vi "4Pi Sample Focus Control.vi"(7 "Calling VI Ref":refnum<vi>) -> ()   [LabVIEW 2021]
uses:
  4Pi Sample Focus Controls/Focus Control.ctl
  4Pi Sample Focus Controls/XY Navigation.ctl
  4Pi Sample Focus Controls/4Pi SFC - Coarse Sample Position.ctl
  <vilib>/Utility/miscctls.llb/LVPointTypeDef.ctl
  Hardware Configuration/Hardware Configuration Controls/Device Function.ctl
  Hardware Configuration/Hardware Configuration Controls/Device Type.ctl
  Device Library/Stages/Stages Controls/Stage Actions.ctl
  Device Library/Shutters/Shutter Controls/Shutter Actions.ctl
panel:
  in  "Unload Sample":bool
  in  "Coarse Sample Z Position":T1
  in  "Engage Upper Objective":bool
  in  "Toggle Shutters":bool
  in  "Lower Shutter":bool
  in  "Upper Shutter":bool
  in  "Quit":bool
  in  "Lower Objective XY":T2
  in  "Upper Objective Focus":T3 {"Step Size (µm)" format="%#_4g"}
  in  "Z Stage Focus":T3 {"Step Size (µm)" format="%#_4g"}
  # "Shutter Control"
  # "step size"
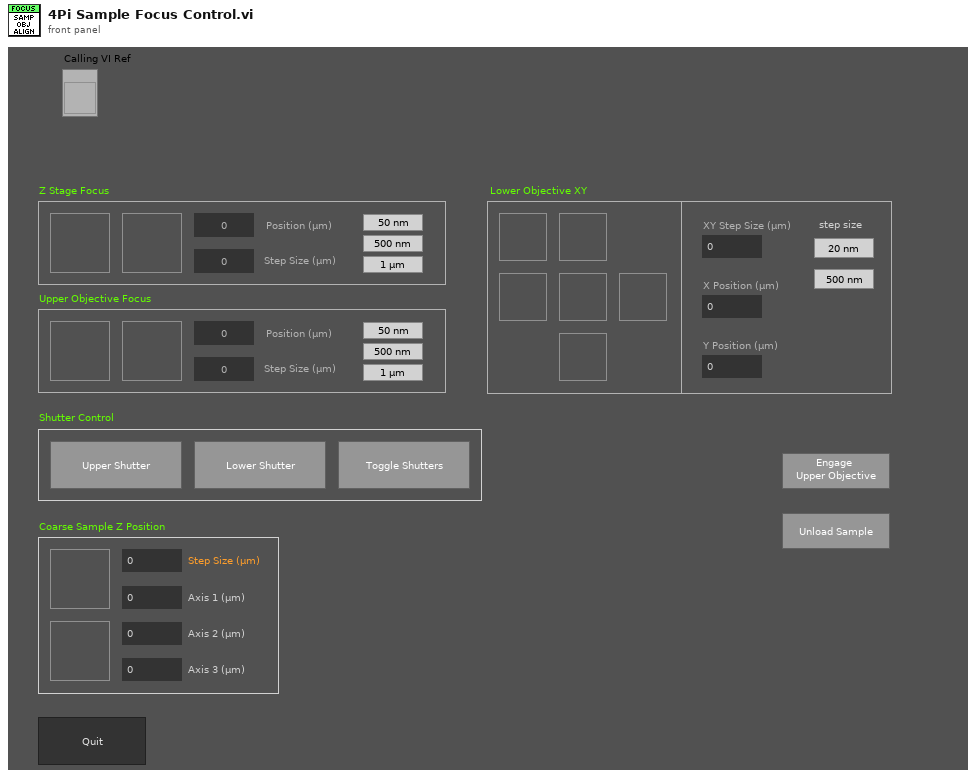
[diagram p1: front panel]
types:
  T1 = typedef "4Pi SFC - Coarse Sample Position.ctl" = cluster{"Z Up":bool, "Z Down":bool, "Step Size (µm)":dbl, "Axis 1 (µm)":dbl, "Axis 2 (µm)":dbl, "Axis 3 (µm)":dbl}
  T2 = typedef "XY Navigation.ctl" = cluster{"Up":bool, "Halt":bool, "Down":bool, "Left":bool, "Right":bool, "Home":bool, "X Position (µm)":dbl, "Y Position (µm)":dbl, "XY Step Size (µm)":dbl, "20nm step":bool, "500nm step":bool}
  T3 = typedef "Focus Control.ctl" = cluster{"Z Up":bool, "Z Down":bool, "Position (µm)":dbl, "Step Size (µm)":dbl, "50nm step":bool, "500nm step":bool, "1µm step":bool}
  T4 = enum16{"Always On", "Always Off", "Off While Running"}
  T5 = typedef "LVPointTypeDef.ctl" = cluster{"Horizontal":i16, "Vertical":i16}
  T6 = typedef "Device Function.ctl" = enum16{"Primary", "Secondary", "Overview", "Wide Field Drift Correction", "642 nm Excitation", "560 nm Excitation", "940 nm Excitation", "546 nm Excitation", "488 nm Excitation", "405 nm Excitation", "Objective Drift Correction", "4Pi Focus Lock", "4Pi Objective Lock", "Objective XY", "Objective Z", "Sample XY", "Sample Coarse Z", "Sample Z", "4Pi Lower", "4Pi Upper", "Em Small", "Em Large", "Ex Small", "Ex Large", "Mojo", "Adj Cavity", "Line Scanning", "Alert"}
  T7 = typedef "Device Type.ctl" = enum16{"AOTF", "Camera", "Deformable Mirror", "Laser", "Flip Mirror", "Shutter", "Stage", "Waveform", "FPGA", "Filter Wheel", "Email"}
  T8 = typedef "Stage Actions.ctl" = enum16{"Get Position", "SERVO OFF", "SERVO ON", "SERVO ON/OFF", "MVR", "MOVE", "HALT", "ONTARGET", "ERROR", "REFERENCE", "INIT", "VELOCITY", "STATUS", "EXIT", "HOME", "ZEROPOS", "NANOPOS", "ANALOG", "QUIT"}
  T9 = typedef "Shutter Actions.ctl" = enum16{"Open", "Close", "Toggle", "Status", "Quit"}
  T10 = cluster{"Z Up":bool, "Z Down":bool, "Position (µm)":bool, "Step Size (µm)":bool, "50nm step":bool, "500nm step":bool, "1µm step":bool}
  T11 = cluster{"Up":bool, "Halt":bool, "Down":bool, "Left":bool, "Right":bool, "Home":bool, "X Position (µm)":bool, "Y Position (µm)":bool, "XY Step Size (µm)":bool, "20nm step":bool, "500nm step":bool}
  T12 = cluster{"Z Up":bool, "Z Down":bool, "Step Size (µm)":bool, "Axis 1 (µm)":bool, "Axis 2 (µm)":bool, "Axis 3 (µm)":bool}
  T13 = typedef "LVRectTypeDef.ctl" = cluster{"Left":i16, "Top":i16, "Right":i16, "Bottom":i16}
  T14 = typedef "LVBoundsTypeDef.ctl" = cluster{"Width":u32, "Height":u32}
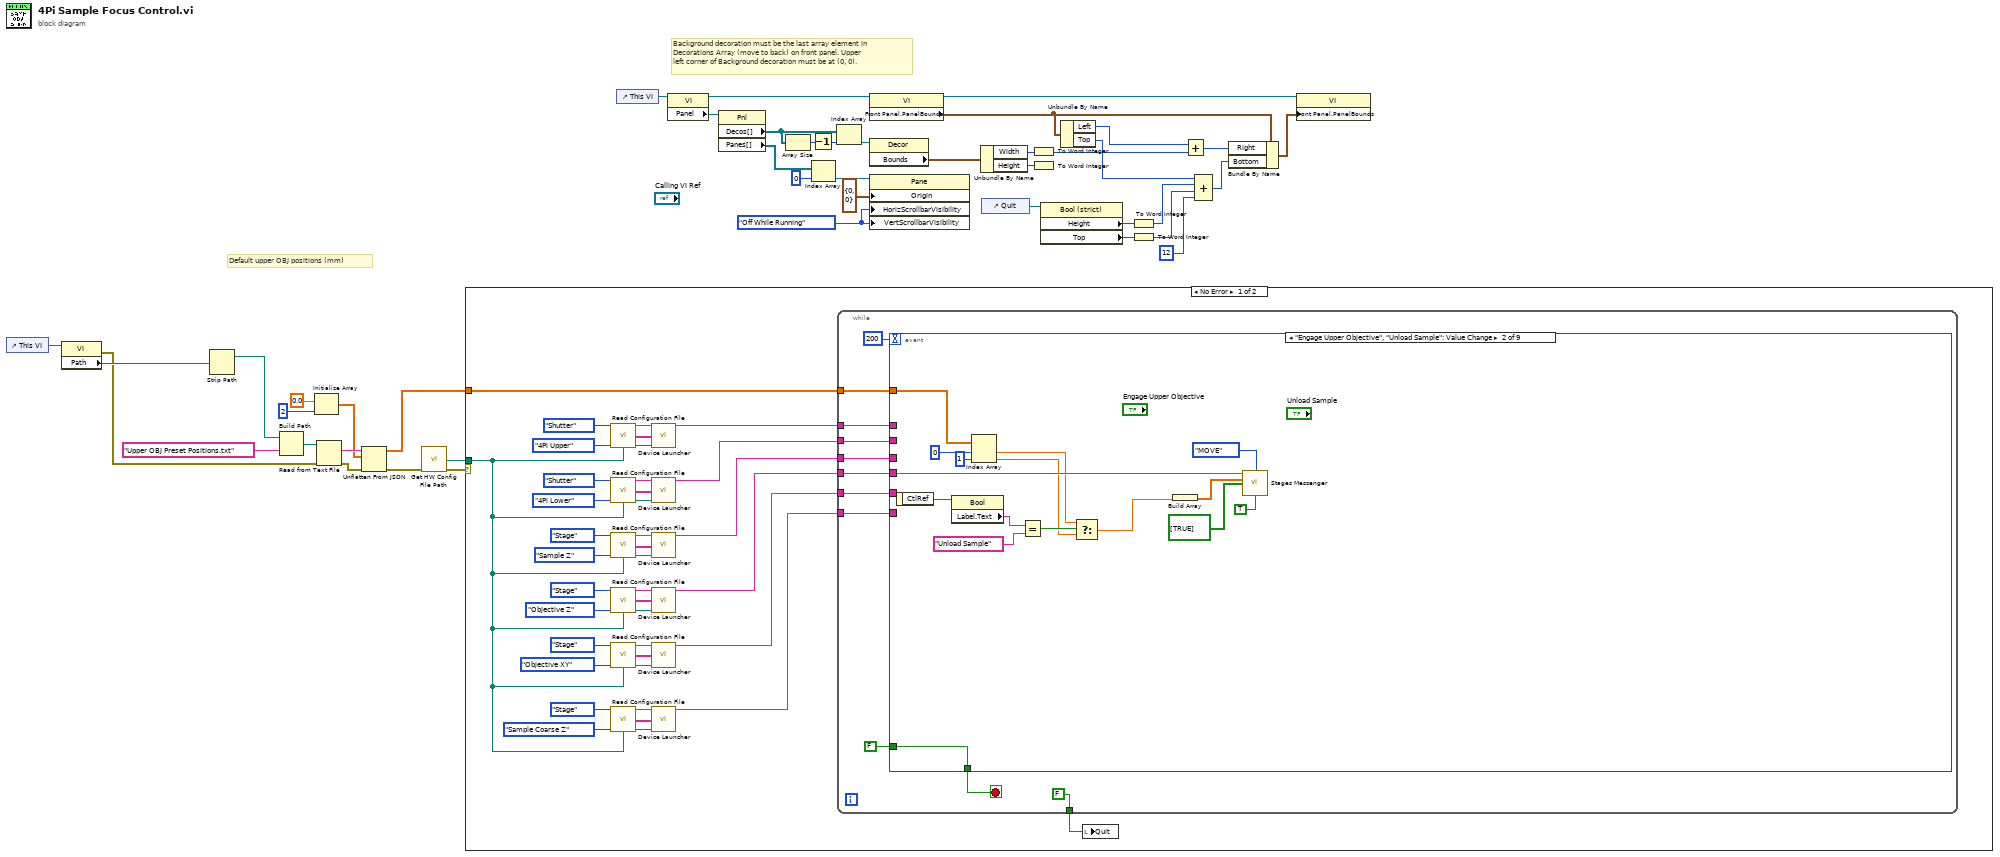
[diagram p0: block diagram]
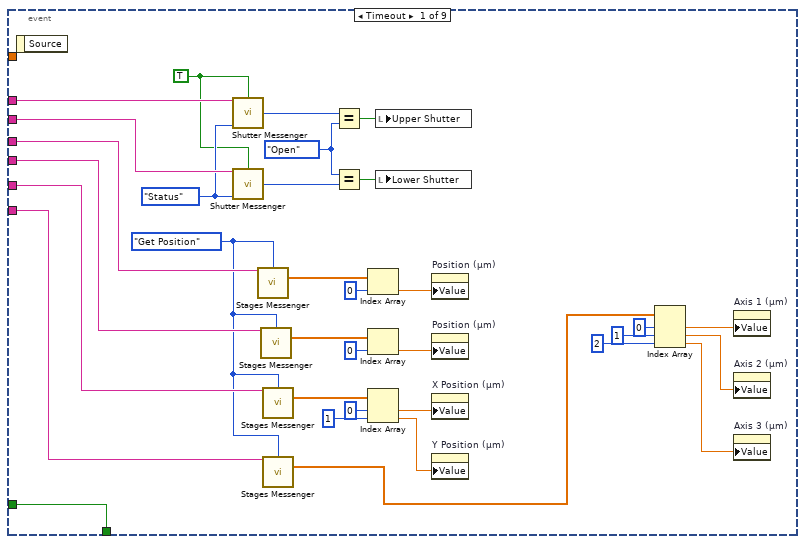
[diagram p2: hidden frame]
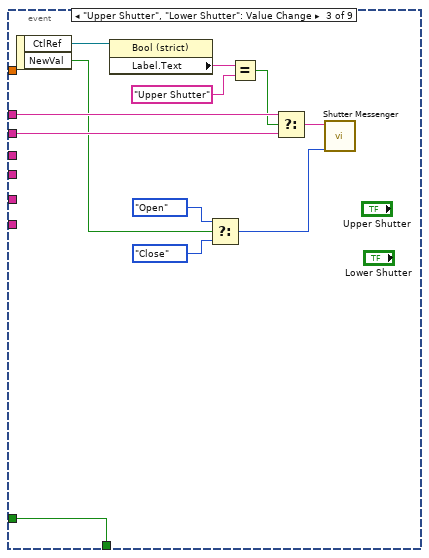
[diagram p3: hidden frame]
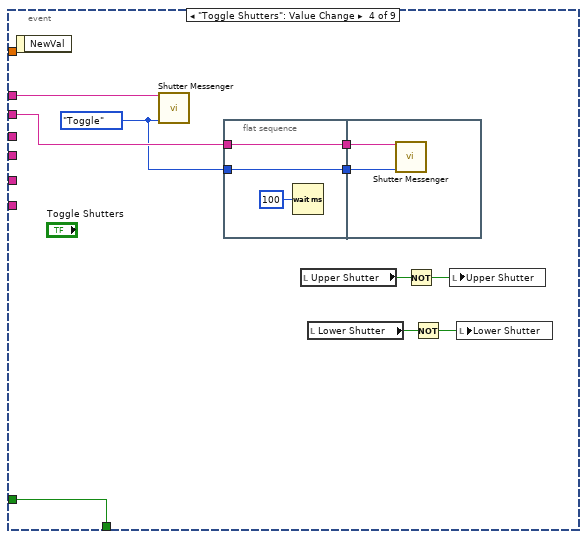
[diagram p4: hidden frame]
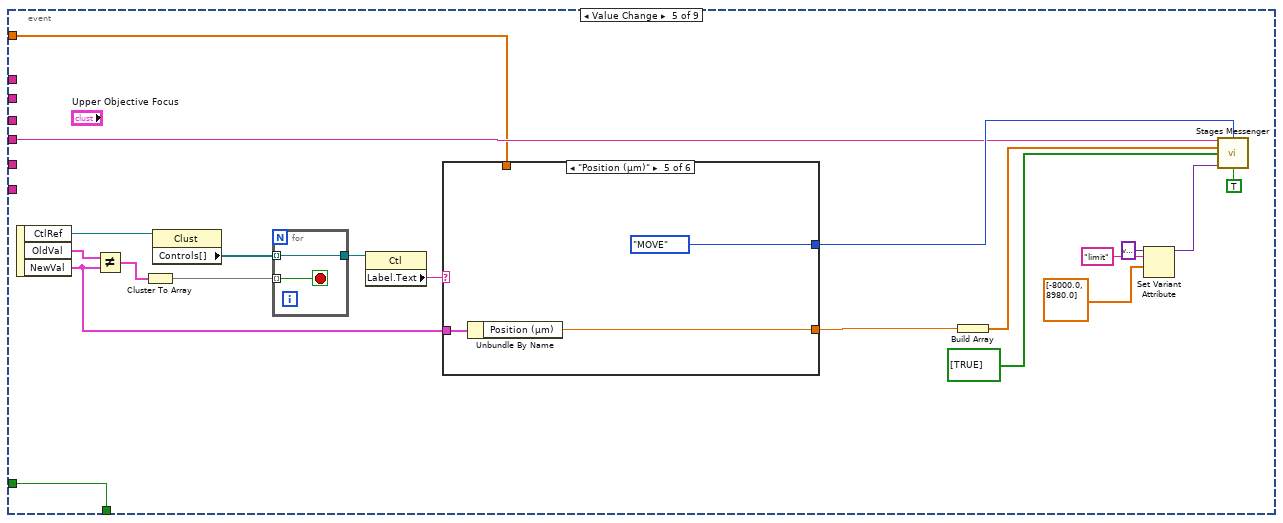
[diagram p5: hidden frame]
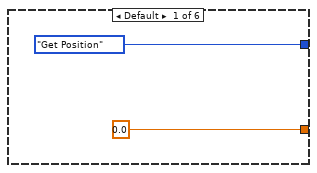
[diagram p6: hidden frame]
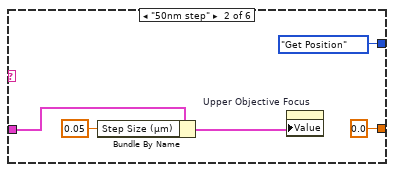
[diagram p7: hidden frame]
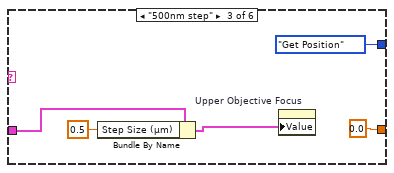
[diagram p8: hidden frame]
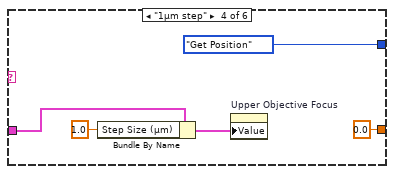
[diagram p9: hidden frame]
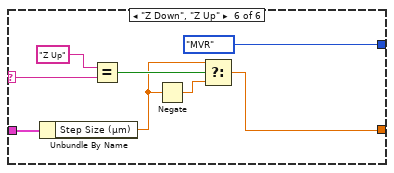
[diagram p10: hidden frame]
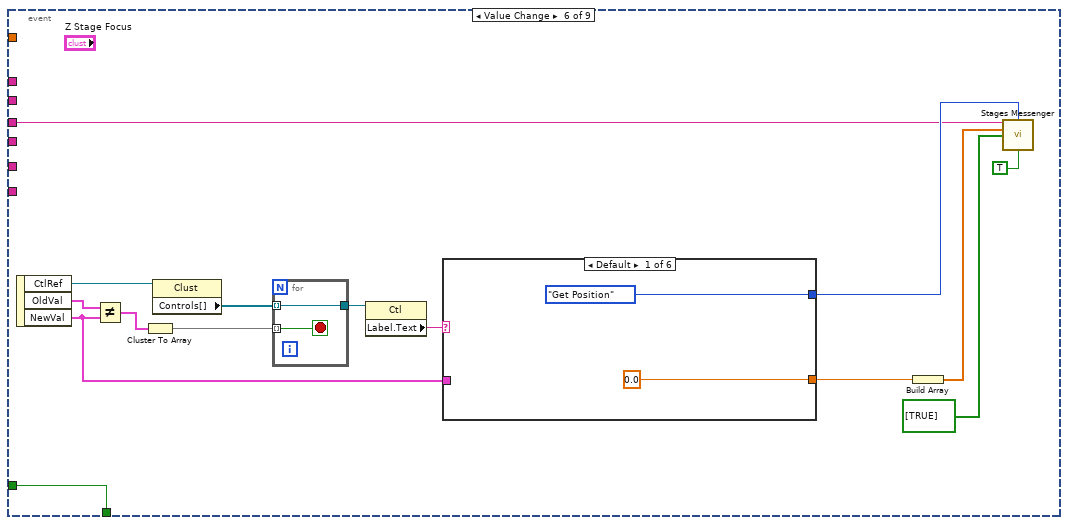
[diagram p11: hidden frame]
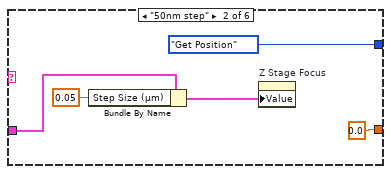
[diagram p12: hidden frame]
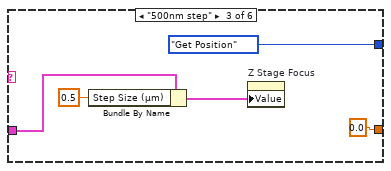
[diagram p13: hidden frame]
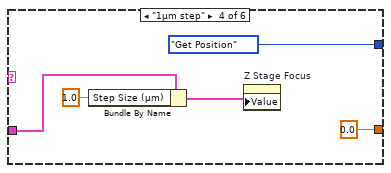
[diagram p14: hidden frame]
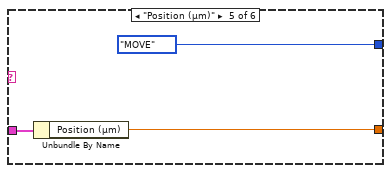
[diagram p15: hidden frame]
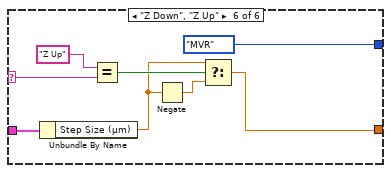
[diagram p16: hidden frame]
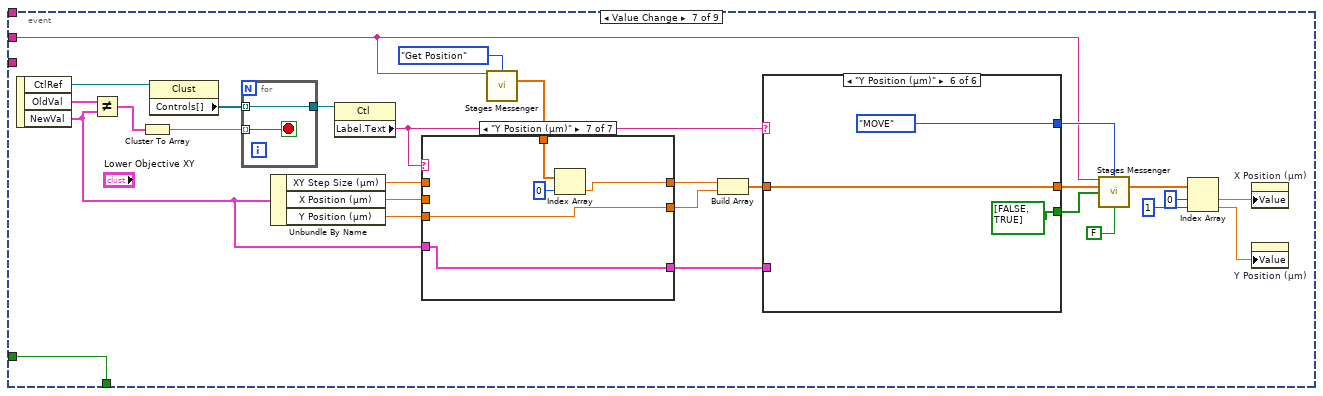
[diagram p17: hidden frame]
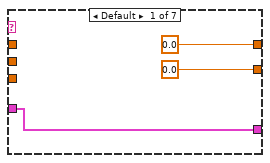
[diagram p18: hidden frame]
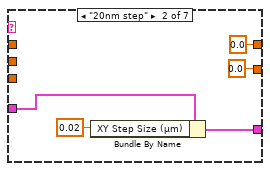
[diagram p19: hidden frame]
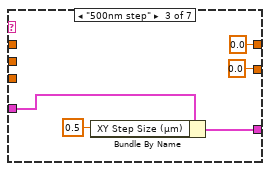
[diagram p20: hidden frame]
diagram:
  w27 = T4."Off While Running" ("Vertical Scrollbar Visibility")
  # "Default upper OBJ positions (mm)"
  # "Background decoration must be the last array element in\nDecorations Array (move to back) on front panel. Upper\nleft corner of Background decoration must be at (0, 0)."
  n1 = control-ref of="This VI"() -> (w13:refnum<vi>)
  n2 = property class="VI"(reference=w13) -> (error out=w3:errorcluster, "Path"=w12:path)  [unwired: 1 in, 1 out]
  n3 = Strip Path(path=w12) -> (stripped path=w11:path)  [unwired: 1 out]
  n4 = Build Path(base path=w11, name or relative path="Upper OBJ Preset Positions.txt") -> (appended path=w9:path)
  n5 = Initialize Array(0.0 ("element"), 2 ("dimension size")) -> (w5:dbl[])
  n6 = Read from Text File(file (use dialog)=w9, error in=w3) -> (text=w8:string, error out=w4:errorcluster)  [unwired: 2 in, 2 out]
  n7 = Unflatten From JSON(JSON string=w8, type and defaults=w5, error in (no error)=w4) -> (value=w1:dbl[], error out=w2:errorcluster)  [unwired: 4 in]
  n8 = call "Get HW Config File Path.vi"("Error"=w2) -> ("File Path"=w15:path, "Error"=w14:errorcluster)  [unwired: 13 in]
  n9 = case shown="No Error" w14 {
    tunnel: w15 -> [w47 _]
    tunnel: w1 -> [w45 _]
    frame No Error {
      n10 = call "Read Configuration File.vi"("Device Type"=Device_Type."Shutter", "Device Function"=Device_Function."4Pi Upper", "Config File Path"=w47) -> ("Unique Notifier Name"=w82:string, "Device Ports/IDs/Channels"=w81:string[], "Device Engine Path"=w80:path)  [unwired: 9 in, 1 out]
      n11 = call "Read Configuration File.vi"("Device Type"=Device_Type."Shutter", "Device Function"=Device_Function."4Pi Lower", "Config File Path"=w47) -> ("Unique Notifier Name"=w73:string, "Device Ports/IDs/Channels"=w74:string[], "Device Engine Path"=w75:path)  [unwired: 9 in, 1 out]
      n12 = call "Read Configuration File.vi"("Device Type"=Device_Type."Stage", "Device Function"=Device_Function."Sample Z", "Config File Path"=w47) -> ("Unique Notifier Name"=w61:string, "Device Ports/IDs/Channels"=w60:string[], "Device Engine Path"=w59:path)  [unwired: 9 in, 1 out]
      n13 = call "Read Configuration File.vi"("Device Type"=Device_Type."Stage", "Device Function"=Device_Function."Objective Z", "Config File Path"=w47) -> ("Unique Notifier Name"=w62:string, "Device Ports/IDs/Channels"=w63:string[], "Device Engine Path"=w64:path)  [unwired: 9 in, 1 out]
      n14 = call "Read Configuration File.vi"("Device Type"=Device_Type."Stage", "Device Function"=Device_Function."Objective XY", "Config File Path"=w47) -> ("Unique Notifier Name"=w71:string, "Device Ports/IDs/Channels"=w70:string[], "Device Engine Path"=w69:path)  [unwired: 9 in, 1 out]
      n15 = call "Read Configuration File.vi"("Device Type"=Device_Type."Stage", "Device Function"=Device_Function."Sample Coarse Z", "Config File Path"=w47) -> ("Unique Notifier Name"=w48:string, "Device Ports/IDs/Channels"=w49:string[], "Device Engine Path"=w50:path)  [unwired: 9 in, 1 out]
      n16 = call "Device Launcher.vi"("Notifier Name"=w82, "Device Ports/IDs/Channels"=w81, "Device Engine Path"=w80) -> ("Notifier Name"=w72:string)  [unwired: 11 in, 1 out]
      n17 = call "Device Launcher.vi"("Notifier Name"=w73, "Device Ports/IDs/Channels"=w74, "Device Engine Path"=w75) -> ("Notifier Name"=w83:string)  [unwired: 11 in, 1 out]
      n18 = call "Device Launcher.vi"("Notifier Name"=w61, "Device Ports/IDs/Channels"=w60, "Device Engine Path"=w59) -> ("Notifier Name"=w56:string)  [unwired: 11 in, 1 out]
      n19 = call "Device Launcher.vi"("Notifier Name"=w62, "Device Ports/IDs/Channels"=w63, "Device Engine Path"=w64) -> ("Notifier Name"=w55:string)  [unwired: 11 in, 1 out]
      n20 = call "Device Launcher.vi"("Notifier Name"=w71, "Device Ports/IDs/Channels"=w70, "Device Engine Path"=w69) -> ("Notifier Name"=w54:string)  [unwired: 11 in, 1 out]
      n21 = call "Device Launcher.vi"("Notifier Name"=w48, "Device Ports/IDs/Channels"=w49, "Device Engine Path"=w50) -> ("Notifier Name"=w46:string)  [unwired: 11 in, 1 out]
      n22 = while {
        tunnel: w72 -> [w93]
        tunnel: w83 -> [w92]
        tunnel: w56 -> [w89]
        tunnel: w55 -> [w88]
        tunnel: w54 -> [w87]
        tunnel: [FALSE] -> w53
        tunnel: w46 -> [w85]
        tunnel: w45 -> [w84]
        stop <- w90 stop-if-true
        n23 = event shown="[1] \"Engage Upper Objective\", \"Unload Sample\": Value Change" {
          selector: _ -> [_ _ _ _ _ _ _ _ _]
          dyn-events: _ -> [_ _ _ _ _ _ _ _ _]
          timeout: 200 -> [_ _ _ _ _ _ _ _ _]
          tunnel: w93 -> [w112 _ w154 w164 _ _ _ _ w410]
          tunnel: w92 -> [w111 _ w153 w163 _ _ _ _ w409]
          tunnel: FALSE -> [w127 w143 w151 w165 w190 w235 w293 w372 _]
          tunnel: [w127 w143 w151 w165 w190 w235 w293 w372 w411] -> w90
          tunnel: w89 -> [w126 _ _ _ _ w221 _ _ _]
          tunnel: w88 -> [w125 w141 _ _ w176 _ _ _ _]
          tunnel: w87 -> [w124 _ _ _ _ _ w268 _ _]
          tunnel: w85 -> [w103 _ _ _ _ _ _ w365 _]
          tunnel: w84 -> [_ w138 _ _ w175 _ _ _ _]
          event Timeout {
            w106 = Shutter_Actions."Open" ("y")
            w109 = TRUE ("Quick Status")
            w110 = Shutter_Actions."Status" ("Action")
            w102 = Stage_Actions."Get Position" ("Actions")
            n24 = event-data() -> ()  [unwired: 1 in, 1 out]
            n25 = call "Shutter Messenger.vi"("Notifier Name"=w112, "Quick Status"=w109, "Action"=w110) -> ("Shutter Status"=w108:T9)  [unwired: 11 in, 1 out]
            n26 = call "Shutter Messenger.vi"("Notifier Name"=w111, "Quick Status"=w109, "Action"=w110) -> ("Shutter Status"=w107:T9)  [unwired: 11 in, 1 out]
            n27 = call "Stages Messenger.vi"("Stage Notifier Name"=w126, "Actions"=w102) -> ("Positions"=w123:dbl[])  [unwired: 9 in, 4 out]
            n28 = call "Stages Messenger.vi"("Stage Notifier Name"=w125, "Actions"=w102) -> ("Positions"=w119:dbl[])  [unwired: 9 in, 4 out]
            n29 = call "Stages Messenger.vi"("Stage Notifier Name"=w124, "Actions"=w102) -> ("Positions"=w118:dbl[])  [unwired: 9 in, 4 out]
            n30 = call "Stages Messenger.vi"("Stage Notifier Name"=w103, "Actions"=w102) -> ("Positions"=w101:dbl[])  [unwired: 9 in, 4 out]
            n31 = Equal?(x=w108, y=w106) -> (x = y?=w105:bool)
            n32 = Equal?(x=w106, y=w107) -> (x = y?=w104:bool)
            n33 = Index Array(array=w123, index=0) -> (element=w113:dbl)
            n34 = Index Array(array=w119, index=0) -> (element=w114:dbl)
            n35 = Index Array(array=w118, index #1=0 ("index"), index #2=1 ("index")) -> (element #1=w116:dbl, element #2=w115:dbl)
            n36 = local write "Upper Shutter"(w105) -> ()
            n37 = local write "Lower Shutter"(w104) -> ()
            n38 = property on="Position (µm)" class="DigNum (strict)"("Value"=w113) -> ()  [unwired: 2 in, 2 out]
            n39 = property on="Position (µm)" class="DigNum (strict)"("Value"=w114) -> ()  [unwired: 2 in, 2 out]
            n40 = property on="X Position (µm)" class="DigNum (strict)"("Value"=w116) -> ()  [unwired: 2 in, 2 out]
            n41 = property on="Y Position (µm)" class="DigNum (strict)"("Value"=w115) -> ()  [unwired: 2 in, 2 out]
            n42 = Index Array(array=w101, index #1=0 ("index"), index #2=1 ("index"), index #3=2 ("index")) -> (element #1=w97:dbl, element #2=w96:dbl, element #3=w95:dbl)
            n43 = property on="Axis 1 (µm)" class="DigNum (strict)"("Value"=w97) -> ()  [unwired: 2 in, 2 out]
            n44 = property on="Axis 2 (µm)" class="DigNum (strict)"("Value"=w96) -> ()  [unwired: 2 in, 2 out]
            n45 = property on="Axis 3 (µm)" class="DigNum (strict)"("Value"=w95) -> ()  [unwired: 2 in, 2 out]
          }
          event "Engage Upper Objective", "Unload Sample": Value Change {
            n46 = event-data() -> ("CtlRef"=w134:refnum<vi>)  [unwired: 1 in]
            n47 = property class="Bool"(reference=w134) -> ("Label.Text"=w133:string)  [unwired: 1 in, 2 out]
            n48 = Index Array(array=w138, index #1=0 ("index"), index #2=1 ("index")) -> (element #1=w130:dbl, element #2=w128:dbl)
            n49 = Equal?(x=w133, y="Unload Sample") -> (x = y?=w131:bool)
            n50 = Select(t=w130, s=w131, f=w128) -> (s? t:f=w129:dbl)
            n51 = Build Array(w129) -> (w136:dbl[])
            n52 = call "Stages Messenger.vi"("Stage Notifier Name"=w141, "Actions"=Stage_Actions."MOVE", "Setpoint"=w136, "Axis"=bool[] [TRUE], "Exit While Busy?"=TRUE) -> ()  [unwired: 6 in, 5 out]
          }
          event "Upper Shutter", "Lower Shutter": Value Change {
            n53 = event-data() -> ("CtlRef"=w155:refnum<vi>, "NewVal"=w152:bool)  [unwired: 1 in]
            n54 = property class="Bool (strict)"(reference=w155) -> ("Label.Text"=w150:string)  [unwired: 1 in, 2 out]
            n55 = Select(t=Shutter_Actions."Open" ("Action"), s=w152, f=Shutter_Actions."Close" ("Action")) -> (s? t:f=w144:T9)
            n56 = Equal?(x=w150, y="Upper Shutter") -> (x = y?=w148:bool)
            n57 = Select(t=w154, s=w148, f=w153) -> (s? t:f=w147:string)
            n58 = call "Shutter Messenger.vi"("Notifier Name"=w147, "Action"=w144) -> ()  [unwired: 12 in, 2 out]
          }
          event "Toggle Shutters": Value Change {
            w162 = Shutter_Actions."Toggle" ("Action")
            n59 = event-data() -> ()  [unwired: 1 in, 1 out]
            n60 = call "Shutter Messenger.vi"("Notifier Name"=w164, "Action"=w162) -> ()  [unwired: 12 in, 2 out]
            n61 = flat-sequence {
              tunnel: w162 -> [w167]
              tunnel: w163 -> [w168]
              tunnel: [w168] -> w157
              tunnel: [w167] -> w156
              tunnel: w157 -> [w170]
              tunnel: w156 -> [w169]
              frame #0 {
                n62 = Wait (ms)(milliseconds to wait=u32 100) -> ()  [unwired: 1 out]
              }
              frame #1 {
                n63 = call "Shutter Messenger.vi"("Notifier Name"=w170, "Action"=w169) -> ()  [unwired: 12 in, 2 out]
              }
            }
            n64 = local read "Upper Shutter"() -> (w161:bool)
            n65 = local read "Lower Shutter"() -> (w160:bool)
            n66 = Not(x=w161) -> (.not. x?=w159:bool)
            n67 = Not(x=w160) -> (.not. x?=w158:bool)
            n68 = local write "Upper Shutter"(w159) -> ()
            n69 = local write "Lower Shutter"(w158) -> ()
          }
          event Value Change {
            n70 = event-data() -> ("CtlRef"=w189:refnum<vi>, "OldVal"=w188:T3, "NewVal"=w182:T3)  [unwired: 1 in]
            n71 = Not Equal?(x=w188, y=w182) -> (x != y?=w186:T10)
            n72 = Cluster To Array(cluster=w186) -> (array=w185:bool[])
            n73 = property class="Clust"(reference=w189) -> ("Controls[]"=w187:refnum<vi>[])  [unwired: 1 in, 2 out]
            n74 = for {
              tunnel: w187 -> [w219] mode=indexing
              tunnel: w185 -> [w220] mode=indexing
              tunnel: [w219] -> w184
              stop <- w220 stop-if-true
            }
            n75 = property class="Ctl"(reference=w184) -> ("Label.Text"=w183:string)  [unwired: 1 in, 2 out]
            n76 = case shown="\"Position (µm)\"" w183 {
              selector: w183 -> [_ _ _ _ _ w213]
              tunnel: w182 -> [_ w195 w200 w205 w209 w211]
              tunnel: [Stage_Actions."Get Position" ("Actions") Stage_Actions."Get Position" ("Actions") Stage_Actions."Get Position" ("Actions") Stage_Actions."Get Position" ("Actions") Stage_Actions."MOVE" ("Actions") Stage_Actions."MVR" ("Actions")] -> w178
              tunnel: [0.0 ("Step Size (µm)") 0.0 ("Step Size (µm)") 0.0 ("Step Size (µm)") 0.0 ("Step Size (µm)") w208 w214] -> w181
              tunnel: w175 -> [_ _ _ _ _ _]
              frame Default {
              }
              frame "50nm step" {
                n77 = Bundle By Name(cluster=w195, "Step Size (µm)"=0.05) -> (w193:T3)
                n78 = property on="Upper Objective Focus" class="Clust"("Value"=w193) -> ()  [unwired: 2 in, 2 out]
              }
              frame "500nm step" {
                n79 = Bundle By Name(cluster=w200, "Step Size (µm)"=0.5) -> (w198:T3)
                n80 = property on="Upper Objective Focus" class="Clust"("Value"=w198) -> ()  [unwired: 2 in, 2 out]
              }
              frame "1µm step" {
                n81 = Bundle By Name(cluster=w205, "Step Size (µm)"=1.0) -> (w203:T3)
                n82 = property on="Upper Objective Focus" class="Clust"("Value"=w203) -> ()  [unwired: 2 in, 2 out]
              }
              frame "Position (µm)" {
                n83 = Unbundle By Name(w209) -> ("Position (µm)"=w208:dbl)
              }
              frame "Z Down", "Z Up" {
                n84 = Unbundle By Name(w211) -> ("Step Size (µm)"=w217:dbl)
                n85 = Equal?(x="Z Up" ("t"), y=w213) -> (x = y?=w218:bool)
                n86 = Negate(x=w217) -> (-x=w216:dbl)
                n87 = Select(t=w217, s=w218, f=w216) -> (s? t:f=w214:dbl)
              }
            }
            n88 = Build Array(w181) -> (w180:dbl[])
            n89 = Set Variant Attribute(Variant=variant ("variant"), name="limit", value=dbl[] [-8000.0, 8980.0] ("Array")) -> (Variant out=w171:variant)  [unwired: 1 in, 2 out]
            n90 = call "Stages Messenger.vi"("Stage Notifier Name"=w176, "Actions"=w178, "Setpoint"=w180, "Axis"=bool[] [TRUE], "Misc"=w171, "Exit While Busy?"=TRUE) -> ()  [unwired: 5 in, 5 out]
          }
          event Value Change {
            n91 = event-data() -> ("CtlRef"=w234:refnum<vi>, "OldVal"=w233:T3, "NewVal"=w227:T3)  [unwired: 1 in]
            n92 = Not Equal?(x=w233, y=w227) -> (x != y?=w231:T10)
            n93 = Cluster To Array(cluster=w231) -> (array=w230:bool[])
            n94 = property class="Clust"(reference=w234) -> ("Controls[]"=w232:refnum<vi>[])  [unwired: 1 in, 2 out]
            n95 = for {
              tunnel: w232 -> [w264] mode=indexing
              tunnel: w230 -> [w265] mode=indexing
              tunnel: [w264] -> w229
              stop <- w265 stop-if-true
            }
            n96 = property class="Ctl"(reference=w229) -> ("Label.Text"=w228:string)  [unwired: 1 in, 2 out]
            n97 = case shown="Default" w228 {
              selector: w228 -> [_ _ _ _ _ w258]
              tunnel: w227 -> [_ w242 w247 w252 w253 w256]
              tunnel: [Stage_Actions."Get Position" ("Actions") Stage_Actions."Get Position" ("Actions") Stage_Actions."Get Position" ("Actions") Stage_Actions."Get Position" ("Actions") Stage_Actions."MOVE" ("Actions") Stage_Actions."MVR" ("Actions")] -> w223
              tunnel: [0.0 ("Step Size (µm)") 0.0 ("Step Size (µm)") 0.0 ("Step Size (µm)") 0.0 ("Step Size (µm)") w254 w259] -> w226
              frame Default {
              }
              frame "50nm step" {
                n98 = Bundle By Name(cluster=w242, "Step Size (µm)"=0.05) -> (w238:T3)
                n99 = property on="Z Stage Focus" class="Clust"("Value"=w238) -> ()  [unwired: 2 in, 2 out]
              }
              frame "500nm step" {
                n100 = Bundle By Name(cluster=w247, "Step Size (µm)"=0.5) -> (w243:T3)
                n101 = property on="Z Stage Focus" class="Clust"("Value"=w243) -> ()  [unwired: 2 in, 2 out]
              }
              frame "1µm step" {
                n102 = Bundle By Name(cluster=w252, "Step Size (µm)"=1.0) -> (w248:T3)
                n103 = property on="Z Stage Focus" class="Clust"("Value"=w248) -> ()  [unwired: 2 in, 2 out]
              }
              frame "Position (µm)" {
                n104 = Unbundle By Name(w253) -> ("Position (µm)"=w254:dbl)
              }
              frame "Z Down", "Z Up" {
                n105 = Unbundle By Name(w256) -> ("Step Size (µm)"=w262:dbl)
                n106 = Equal?(x="Z Up" ("t"), y=w258) -> (x = y?=w263:bool)
                n107 = Negate(x=w262) -> (-x=w261:dbl)
                n108 = Select(t=w262, s=w263, f=w261) -> (s? t:f=w259:dbl)
              }
            }
            n109 = Build Array(w226) -> (w225:dbl[])
            n110 = call "Stages Messenger.vi"("Stage Notifier Name"=w221, "Actions"=w223, "Setpoint"=w225, "Axis"=bool[] [TRUE], "Exit While Busy?"=TRUE) -> ()  [unwired: 6 in, 5 out]
          }
          event Value Change {
            n111 = event-data() -> ("CtlRef"=w289:refnum<vi>, "OldVal"=w288:T2, "NewVal"=w270:T2)  [unwired: 1 in]
            n112 = Not Equal?(x=w288, y=w270) -> (x != y?=w292:T11)
            n113 = Cluster To Array(cluster=w292) -> (array=w291:bool[])
            n114 = property class="Clust"(reference=w289) -> ("Controls[]"=w287:refnum<vi>[])  [unwired: 1 in, 2 out]
            n115 = for {
              tunnel: w287 -> [w357] mode=indexing
              tunnel: w291 -> [w358] mode=indexing
              tunnel: [w357] -> w290
              stop <- w358 stop-if-true
            }
            n116 = Unbundle By Name(w270) -> ("XY Step Size (µm)"=w281:dbl, "X Position (µm)"=w280:dbl, "Y Position (µm)"=w279:dbl)
            n117 = property class="Ctl"(reference=w290) -> ("Label.Text"=w282:string)  [unwired: 1 in, 2 out]
            n118 = call "Stages Messenger.vi"("Stage Notifier Name"=w268, "Actions"=Stage_Actions."Get Position") -> ("Positions"=w266:dbl[])  [unwired: 9 in, 4 out]
            n119 = case shown="\"Y Position (µm)\"" w282 {
              tunnel: w281 -> [_ _ _ w310 w315 _ _]
              tunnel: w280 -> [_ _ _ _ _ w322 _]
              tunnel: w279 -> [_ _ _ _ _ _ w327]
              tunnel: [0.0 ("Y Position (µm)") 0.0 ("X Position (µm)") 0.0 ("X Position (µm)") w309 w314 w322 w323] -> w278
              tunnel: [0.0 0.0 ("Y Position (µm)") 0.0 ("Y Position (µm)") w308 w314 w318 w327] -> w271
              tunnel: w270 -> [w294 w301 w306 w307 w313 w321 w326]
              tunnel: [w294 w297 w302 w307 w313 w321 w326] -> w269
              tunnel: w266 -> [_ _ _ _ _ w320 w325]
              frame Default {
              }
              frame "20nm step" {
                n120 = Bundle By Name(cluster=w301, "XY Step Size (µm)"=0.02) -> (w297:T2)
              }
              frame "500nm step" {
                n121 = Bundle By Name(cluster=w306, "XY Step Size (µm)"=0.5) -> (w302:T2)
              }
              frame "Down", "Up" {
                n122 = Square Root(x=2.0) -> (sqrt(x)=w311:dbl)
                n123 = Divide(x=w310, y=w311) -> (x/y=w309:dbl)
                n124 = Negate(x=w309) -> (-x=w308:dbl)
              }
              frame "Left", "Right" {
                n125 = Square Root(x=2.0) -> (sqrt(x)=w316:dbl)
                n126 = Divide(x=w315, y=w316) -> (x/y=w314:dbl)
              }
              frame "X Position (µm)" {
                n127 = Index Array(array=w320, index=1) -> (element=w318:dbl)
              }
              frame "Y Position (µm)" {
                n128 = Index Array(array=w325, index=0) -> (element=w323:dbl)
              }
            }
            n129 = Build Array(w278, w271) -> (w286:dbl[])
            n130 = case shown="\"Y Position (µm)\"" w282 {
              selector: w282 -> [_ _ w342 w347 _ _]
              tunnel: w286 -> [_ _ w339 w346 w352 w355]
              tunnel: [dbl[] [0.0, 0.0] dbl[] [0.0, 0.0] w335 w343 w352 w355] -> w285
              tunnel: [bool[] [TRUE, TRUE] bool[] [TRUE, TRUE] bool[] [TRUE, TRUE] bool[] [TRUE, TRUE] bool[] [TRUE] bool[] [FALSE, TRUE]] -> w284
              tunnel: [Stage_Actions."Get Position" ("Actions") Stage_Actions."MOVE" ("Actions") Stage_Actions."MVR" ("Actions") Stage_Actions."MVR" ("Actions") Stage_Actions."MOVE" ("Actions") Stage_Actions."MOVE" ("Actions")] -> w283
              tunnel: w269 -> [w328 _ _ _ _ _]
              frame Default {
                n131 = property on="Lower Objective XY" class="Clust"("Value"=w328) -> ()  [unwired: 2 in, 2 out]
              }
              frame "Home" {
              }
              frame "Down", "Up" {
                n132 = Negate(x=w339) -> (-x=w340:dbl[])
                n133 = Equal?(x=w342, y="Up") -> (x = y?=w338:bool)
                n134 = Select(t=w340, s=w338, f=w339) -> (s? t:f=w335:dbl[])
              }
              frame "Left", "Right" {
                n135 = Negate(x=w346) -> (-x=w349:dbl[])
                n136 = Equal?(x=w347, y="Right") -> (x = y?=w348:bool)
                n137 = Select(t=w349, s=w348, f=w346) -> (s? t:f=w343:dbl[])
              }
              frame "X Position (µm)" {
              }
              frame "Y Position (µm)" {
              }
            }
            n138 = call "Stages Messenger.vi"("Stage Notifier Name"=w268, "Actions"=w283, "Setpoint"=w285, "Axis"=w284, "Exit While Busy?"=FALSE) -> ("Positions"=w272:dbl[])  [unwired: 6 in, 4 out]
            n139 = Index Array(array=w272, index #1=0 ("index"), index #2=1 ("index")) -> (element #1=w274:dbl, element #2=w273:dbl)
            n140 = property on="X Position (µm)" class="DigNum (strict)"("Value"=w274) -> ()  [unwired: 2 in, 2 out]
            n141 = property on="Y Position (µm)" class="DigNum (strict)"("Value"=w273) -> ()  [unwired: 2 in, 2 out]
          }
          event Value Change {
            n142 = event-data() -> ("CtlRef"=w368:refnum<vi>, "OldVal"=w367:T1, "NewVal"=w363:T1)  [unwired: 1 in]
            n143 = Not Equal?(x=w367, y=w363) -> (x != y?=w371:T12)
            n144 = Cluster To Array(cluster=w371) -> (array=w370:bool[])
            n145 = property class="Clust"(reference=w368) -> ("Controls[]"=w366:refnum<vi>[])  [unwired: 1 in, 2 out]
            n146 = for {
              tunnel: w366 -> [w406] mode=indexing
              tunnel: w370 -> [w407] mode=indexing
              tunnel: [w406] -> w369
              stop <- w407 stop-if-true
            }
            n147 = property class="Ctl"(reference=w369) -> ("Label.Text"=w364:string)  [unwired: 1 in, 2 out]
            n148 = case shown="\"Z Down\", \"Z Up\"" w364 {
              selector: w364 -> [_ w384 w390]
              tunnel: w363 -> [_ w386 w395]
              tunnel: [dbl[] [0.0, 0.0, 0.0] w378 w391] -> w359
              tunnel: [bool[] [FALSE, FALSE, FALSE] bool[] [TRUE, TRUE, TRUE] w389] -> w360
              tunnel: [Stage_Actions."Get Position" ("Actions") Stage_Actions."MVR" ("Actions") Stage_Actions."MOVE" ("Actions")] -> w361
              frame Default {
              }
              frame "Z Down", "Z Up" {
                n149 = Unbundle By Name(w386) -> ("Step Size (µm)"=w381:dbl)
                n150 = Equal?(x=w384, y="Z Down") -> (x = y?=w382:bool)
                n151 = Negate(x=w381) -> (-x=w380:dbl)
                n152 = Select(t=w380, s=w382, f=w381) -> (s? t:f=w379:dbl)
                n153 = Initialize Array(w379, 3 ("dimension size")) -> (w378:dbl[])
              }
              frame "Axis 1 (µm)", "Axis 2 (µm)", "Axis 3 (µm)" {
                n154 = Unbundle By Name(w395) -> ("Axis 1 (µm)"=w394:dbl, "Axis 2 (µm)"=w392:dbl, "Axis 3 (µm)"=w393:dbl)
                n155 = for {
                  N: 3 -> [_]
                  tunnel: w390 -> [w397]
                  tunnel: [w396] -> w389 mode=indexing
                  i -> [w405]
                  n156 = Increment(x=w405) -> (x+1=w399:i32)
                  n157 = Format Into String(format string="%d", w399) -> (resulting string=w402:string)  [unwired: 2 in, 1 out]
                  n158 = call <vilib>:"Space Constant.vi"() -> ("String"=w401:string)
                  n159 = Concatenate Strings("Axis" ("initial string"), w401, w402, w401, "(µm)" ("initial string")) -> (w398:string)
                  n160 = Equal?(x=w398, y=w397) -> (x = y?=w396:bool)
                }
                n161 = Build Array(w394, w392, w393) -> (w391:dbl[])
              }
            }
            n162 = call "Stages Messenger.vi"("Stage Notifier Name"=w365, "Actions"=w361, "Setpoint"=w359, "Axis"=w360, "Exit While Busy?"=TRUE) -> ()  [unwired: 6 in, 5 out]
          }
          event "Quit": Value Change {
            n163 = event-data() -> ("NewVal"=w411:bool)  [unwired: 1 in]
            n164 = Build Array(w410, w409) -> (w408:string[])
            n165 = for {
              tunnel: w408 -> [w413] mode=indexing
              n166 = call "Shutter Messenger.vi"("Notifier Name"=w413, "Action"=Shutter_Actions."Close") -> ()  [unwired: 12 in, 2 out]
            }
          }
        }
      }
      n167 = local write "Quit"(w53) -> ()
    }
    frame Error {
      n168 = control-ref of="This VI"() -> (w419:refnum<vi>)
      n169 = property class="VI"(reference=w419) -> ("Name"=w417:string)  [unwired: 1 in, 2 out]
      n170 = Concatenate Strings("Error in ", w417, "\r", "No Config File") -> (w414:string)
      n171 = One Button Dialog(message=w414) -> ()  [unwired: 1 in, 1 out]
    }
  }
  n172 = control-ref of="This VI"() -> (w20:refnum<vi>)
  n173 = property class="VI"(reference=w20) -> (reference out=w28:refnum<vi>, "Panel"=w21:refnum<vi>)  [unwired: 1 in, 1 out]
  n174 = property class="Pnl"(reference=w21) -> ("Decos[]"=w19:refnum<vi>[], "Panes[]"=w24:refnum<vi>[])  [unwired: 1 in, 2 out]
  n175 = Array Size(array=w19) -> (size(s)=w17:i32)
  n176 = Decrement(x=w17) -> (x-1=w18:i32)
  n177 = Index Array(array=w24, index=0) -> (element=w23:refnum<vi>)
  n178 = Index Array(array=w19, index=w18) -> (element=w26:refnum<vi>)
  n179 = property class="VI"(reference=w28) -> (reference out=w30:refnum<vi>, "Front Panel.PanelBounds"=w31:T13)  [unwired: 1 in, 1 out]
  n180 = property class="Decor"(reference=w26) -> ("Bounds"=w29:T14)  [unwired: 1 in, 2 out]
  n181 = property class="Pane"(reference=w23, "Origin"=T5 {"Horizontal"=0, "Vertical"=0}, "HorizScrollbarVisibility"=w27, "VertScrollbarVisibility"=w27) -> ()  [unwired: 1 in, 2 out]
  n182 = Unbundle By Name(w29) -> ("Width"=w34:u32, "Height"=w37:u32)
  n183 = control-ref of="Quit"() -> (w16:refnum<vi>)
  n184 = To Word Integer(number=w34) -> (16bit integer=w36:i16)
  n185 = To Word Integer(number=w37) -> ()  [unwired: 1 out]
  n186 = property class="Bool (strict)"(reference=w16) -> ("Height"=w39:u32, "Top"=w40:i32)  [unwired: 1 in, 2 out]
  n187 = Unbundle By Name(w31) -> ("Left"=w33:i16, "Top"=w44:i16)
  n188 = To Word Integer(number=w39) -> (16bit integer=w42:i16)
  n189 = To Word Integer(number=w40) -> (16bit integer=w43:i16)
  n190 = Add(x=w33, y=w36) -> (x+y=w35:i16)
  n191 = Compound Arithmetic op=ADD(w44, w42, w43, i16 12 ("y")) -> (w38:i16)
  n192 = Bundle By Name(cluster=w31, "Right"=w35, "Bottom"=w38) -> (w32:T13)
  n193 = property class="VI"(reference=w30, "Front Panel.PanelBounds"=w32) -> ()  [unwired: 1 in, 2 out]
